vi "I2C Read Reg Block.vi"(8 "error in (no error)":errorcluster, 9 "Size":i32=1, 10 "Register":i32, 11 "I2C Device":T1) -> (0 "error out":errorcluster, 2 "Values":u8[](array[numeric]), 3 "I2C Device out":T1)   [LabVIEW 2020, in "wiringPi.lvlib"]
doc: "<b>_______________________________________________________________</b>\n** Author: Juan José Villacorta\n** LabVIEW wrapper for C library <b> wiringPi </b>,\n** https://github.com/WiringPi/WiringPi\n<b>_______________________________________________________________</b>\n/*\n * Read a block of data from a register on the device\n**********************************************************************************\n*/"
uses:
  wiringPi.lvlib
  Type Defs/I2C Device.ctl
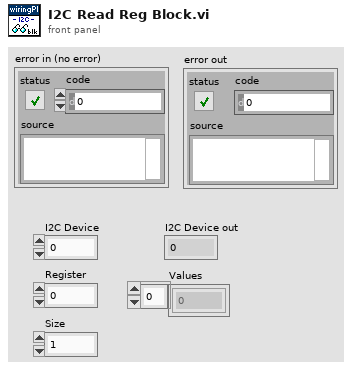
[diagram p1: front panel]
types:
  T1 = typedef "wiringPi.lvlib/I2C Device.ctl" = i32
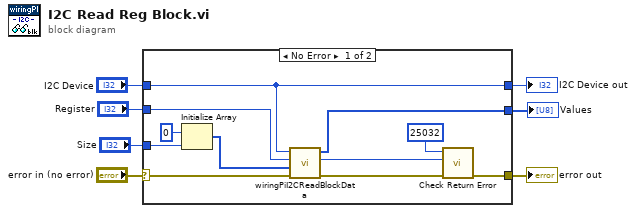
[diagram p0: block diagram]
diagram:
  n1 = case shown="No Error" "error in (no error)" {
    selector: "error in (no error)" -> [w17 w20]
    tunnel: [w18 w20] -> w6
    tunnel: "I2C Device" -> [w15 w19]
    tunnel: [w15 w19] -> w5
    tunnel: "Register" -> [w12 _]
    tunnel: "Size" -> [w11 _]
    tunnel: [w8 _] -> w1
    frame No Error {
      n2 = Initialize Array(u8 0 ("element"), w11) -> (w10:u8[])
      n3 = call "wiringPiI2CReadBlockData.vi"("error in (no error)"=w17, "values"=w10, "reg"=w12, "devID"=w15) -> ("error out"=w16:errorcluster, "return"=w14:i32, "values readed"=w8:u8[])  [unwired: 5 in]
      n4 = call "Check Return Error.vi"("error in (no error)"=w16, "Return code"=w14, "Error number"=25032) -> ("error out"=w18:errorcluster)  [unwired: 8 in]
    }
    frame Error {
    }
  }
  "error out" <- w6
  "I2C Device out" <- w5
  "Values" <- w1
